vi "Refresh Values.vi"(8 "error in (no error)":errorcluster, 11 "PluginGUI in":refnum<class "PluginGUI.lvclass">) -> (0 "error out":errorcluster, 3 "PluginGUI out":refnum<class "PluginGUI.lvclass">)   [LabVIEW 2020, in "VolatusGUI.lvlib" / "PluginGUI.lvclass"]
uses:
  PluginGUI.lvclass
  C:/dev/lv20CE/relink/lv-volatus/Volatus/Module/Module.lvclass
  Volatus/Module/Module.lvclass/Module.ctl
  PluginGUI.lvclass/PluginGUI.ctl
  GUI Element/GUI Element.lvclass/GUI Element.ctl
  GUI Element/GUI Element.lvclass
  Volatus/Module/Module.lvclass
  C:/dev/lv20CE/relink/lv-volatus/VolatusGUI/PluginGUI/PluginGUI.lvclass
  Volatus/VolatusAPI/VolatusAPI.lvclass
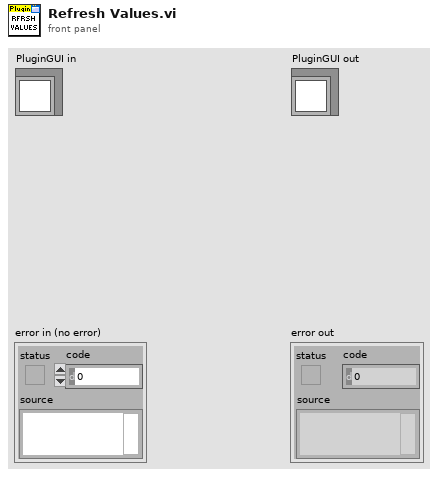
[diagram p1: front panel]
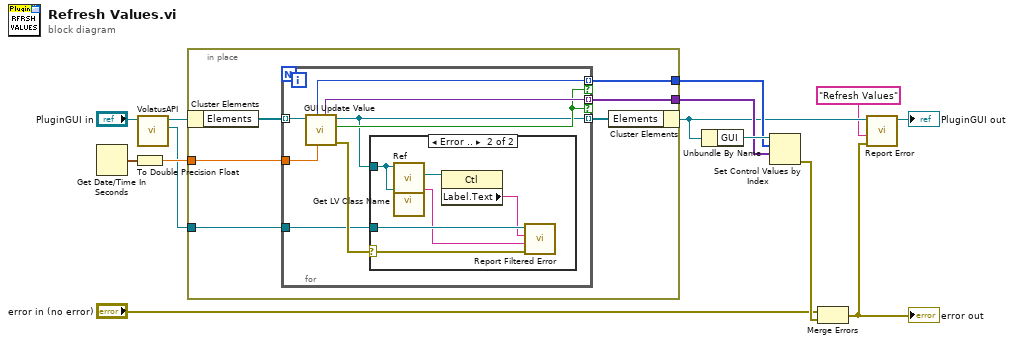
[diagram p0: block diagram]
diagram:
  n1 = Get Date/Time In Seconds() -> (seconds since 1Jan1904=w6:timestamp)
  n2 = To Double Precision Float(number=w6) -> (double precision float=w5:dbl)
  n3 = call "VolatusAPI.vi"("Module in"="PluginGUI in") -> ("VolatusAPI"=w2:refnum<class "VolatusAPI.lvclass">, "Module out"=w3:refnum<class "PluginGUI.lvclass">)  [unwired: 9 in]
  n4 = in-place {
    in-place-border: [w20] -> w13
    in-place-border: [w19] -> w12
    in-place-border: w5 -> [w16]
    in-place-border: w2 -> [w15]
    n5 = in-place-cluster #1(w3) -> ("Elements"=w18:refnum<class "GUI Element.lvclass">[])
    n6 = for {
      tunnel: [w28] -> w20 mode=indexing if=w26
      tunnel: [w27] -> w19 mode=indexing if=w26
      tunnel: w18 -> [w25] mode=indexing
      tunnel: [w21] -> w17 mode=indexing
      tunnel: w16 -> [w24]
      tunnel: w15 -> [w22]
      n7 = call "GUI Update Value.vi"("Time"=w24, "GUI Element in"=w25) -> ("error out"=w23:errorcluster, "Update"=w26:bool, "GUI Element out"=w21:refnum<class "GUI Element.lvclass">, "Value"=w27:variant, "Control Index"=w28:i32)  [unwired: 5 in]
      n8 = case shown="Error .." w23 {
        selector: w23 -> [_ w34]
        tunnel: w22 -> [_ w33]
        tunnel: w21 -> [_ w32]
        frame No Error {
        }
        frame Error {
          n9 = call "Ref.vi"("GUI Element in"=w32) -> ("Ref"=w31:refnum<vi>)  [unwired: 9 in, 1 out]
          n10 = call <vilib>:"Get LV Class Name.vi"("object"=w32) -> ("class name"=w29:string)  [unwired: 9 in, 1 out]
          n11 = property class="Ctl"(reference=w31) -> ("Label.Text"=w30:string)  [unwired: 1 in, 2 out]
          n12 = call "Report Filtered Error.vi"("error in (no error)"=w34, "Message"=w29, "Context"=w30, "VolatusAPI in"=w33) -> ()  [unwired: 6 in, 2 out]
        }
      }
    }
    n13 = in-place-cluster #1("Elements"=w17) -> (w8:refnum<class "PluginGUI.lvclass">)
  }
  n14 = Unbundle By Name(w8) -> ("GUI"=w14:refnum<vi>)
  n15 = Set Control Values by Index(0:w14, 1:w13, 2:w12) -> (11:w11:errorcluster)  [unwired: 1 in]
  n16 = Merge Errors("error in (no error)", w11) -> (w10:errorcluster)
  "error out" <- w10
  n17 = call "Report Error.vi"("error in (no error)"=w10, "Message (None)"="Refresh Values", "Module in"=w8) -> ("Module in"=→"PluginGUI out":refnum<class "PluginGUI.lvclass">)  [unwired: 7 in, 1 out]
